vi "Check_station.vi"(8 "error in":errorcluster, 11 "Serial no":string) -> (0 "error out":errorcluster, 3 "Result":bool)   [LabVIEW 2021]
panel:
  out "offset past match":i32
  out "standard output":string
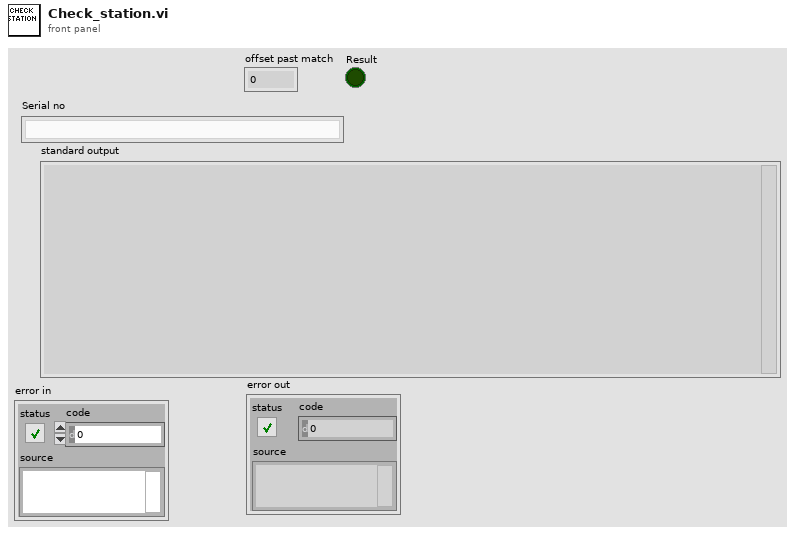
[diagram p1: front panel]
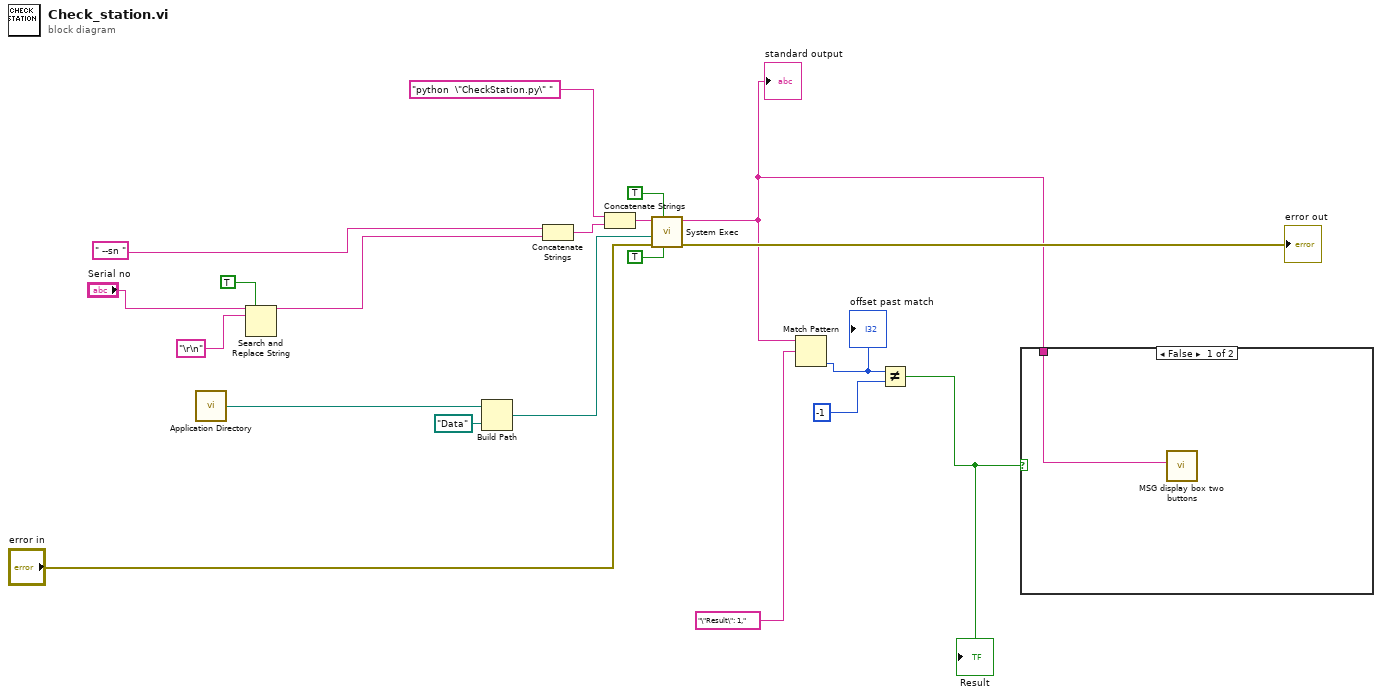
[diagram p0: block diagram]
diagram:
  n1 = call <vilib>:"Application Directory.vi"() -> ("Application Directory"=w14:path)
  n2 = Search and Replace String(replace all?=TRUE ("replace all? (F)"), input string="Serial no", search string="\r\n") -> (result string=w2:string)  [unwired: 5 in, 3 out]
  n3 = Build Path(base path=w14, name or relative path=path "Data") -> (appended path=w13:path)
  n4 = Concatenate Strings(" --sn " ("string"), w2) -> (w18:string)
  n5 = Concatenate Strings("python  \"CheckStation.py\" " ("command line"), w18) -> (w19:string)
  n6 = call <vilib>:"System Exec.vi"("run minimized? (F)"=TRUE, "wait until completion? (T)"=TRUE, "error in (no error)"="error in", "working directory"=w13, "command line"=w19) -> ("error out"=→"error out":errorcluster, "standard output"=w5:string)  [unwired: 3 in, 2 out]
  "standard output" <- w5
  n7 = Match Pattern(string=w5, regular expression="\"Result\": 1,") -> (offset past match=w9:i32)  [unwired: 1 in, 3 out]
  "offset past match" <- w9
  n8 = Not Equal?(x=w9, y=-1) -> (x != y?=w7:bool)
  "Result" <- w7
  n9 = case shown="False" w7 {
    tunnel: w5 -> [w21 _]
    frame False {
      n10 = call "MSG display box two buttons.vi"("input string"=w21) -> ()  [unwired: 8 in, 3 out]
    }
    frame True {
    }
  }
